vi "New File Handler 2.vi"   [LabVIEW 2018, in "GLog.lvlib" / "File Handler.lvclass"]
uses:
  File Handler.lvclass
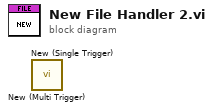
[diagram p0: block diagram]
diagram:
  n1 = call "New (Multi Trigger).vi"() -> ()  [unwired: 9 in, 3 out]
  n2 = call "New (Single Trigger).vi"() -> ()  [unwired: 9 in, 3 out]
